vi "RemoteVI Translate Input.vi"(0 "kind":T2(ring), 1 "msg":u32, 2 "x":i32, 3 "y":i32, 4 "wParam":u64, 5 "lParam":i64, 6 "geo":T1, 7 "tracking in":bool, 8 "popup":bool) -> (20 "posts":cluster{"msg":u32, "wParam":u64, "lParam":i64}[](array[cluster]), 21 "tracking out":bool, 22 "cursor":cluster{"move?":bool, "x":i32, "y":i32})   [LabVIEW 2020, in "RemoteVI.lvlib"]
doc: "Turns one parsed client input message (the outputs of RemoteVI Parse Input.vi) into the Win32 messages the server posts to the panel window (docs/protocol.md section 4). Only the allowed messages of section 4.3 produce posts; anything else - ack, invalid, WM_CLOSE, WM_SYSKEYDOWN - gives an empty posts array and leaves tracking unchanged. WM_CHAR becomes three posts: WM_KEYDOWN(0xE8,1), WM_CHAR(wParam,1), WM_KEYUP(0xE8,0xC0000001). Other key messages pass through, except that a WM_KEYDOWN/WM_KEYUP whose lParam has no scan code (bits 16-23 zero - the browser client sends none) gets the key's set-1 scan code from the table below (LabVIEW lost the arrow key of a posted Shift + Right when both had scan code 0, measured). A double click (WM_xBUTTONDBLCLK) is posted as a second WM_xBUTTONDOWN: LabVIEW's panel window class has no CS_DBLCLKS, so Windows sends it two downs and LabVIEW ignores a posted DBLCLK (measured with a listbox Double Click event). Mouse lParam = ((y and 0xFFFF) shl 16) or (x and 0xFFFF) of CLIENT coordinates (screen point minus client origin) or of SCREEN coordinates (frame origin plus x/y - x and y are frame pixels, the frame being the window below its title bar): the wheel always uses screen; a button-down uses client and starts tracking; a button-up uses screen while tracking in is TRUE, else client, and ends tracking; a move uses screen while tracking in is TRUE, else client. The server passes as tracking in whether LabVIEW tracks the press right now - its UI thread holds the mouse capture (RemoteVI Mouse Captured.vi), read after LabVIEW handled the button-down. LabVIEW reads moves and the button-up as SCREEN coordinates only while it tracks (latched buttons, sliders, text selection, graph drags); a switch-when-pressed does not track and lost a screen-coordinate button-up (measured). While a LabVIEW popup is open (popup TRUE) only BUTTON messages are posted: with SCREEN coordinates, and cursor asks the caller to move the host cursor to that screen point just for the click (popup menus read the real cursor); tracking follows the same button rules. Moves and the wheel are DROPPED while a popup is open (no posts, tracking unchanged, no cursor), so the host cursor stays where the host user left it. Key messages are unaffected by popup. Pure function, cannot fail. Reference: translateInput() in tools\\lib\\input.mjs."
uses:
  RemoteVI.lvlib
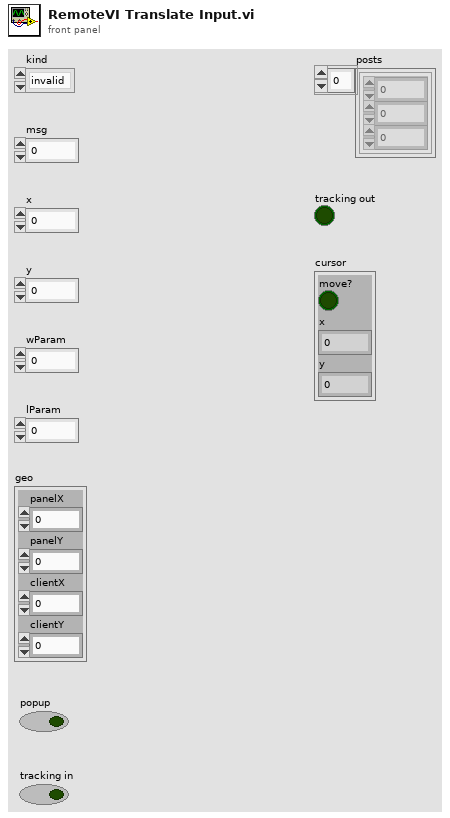
[diagram p1: front panel]
types:
  T1 = cluster{"panelX":i32, "panelY":i32, "clientX":i32, "clientY":i32}
  T2 = enum16{"invalid", "mouse", "key", "ack", "close", "splitter"}
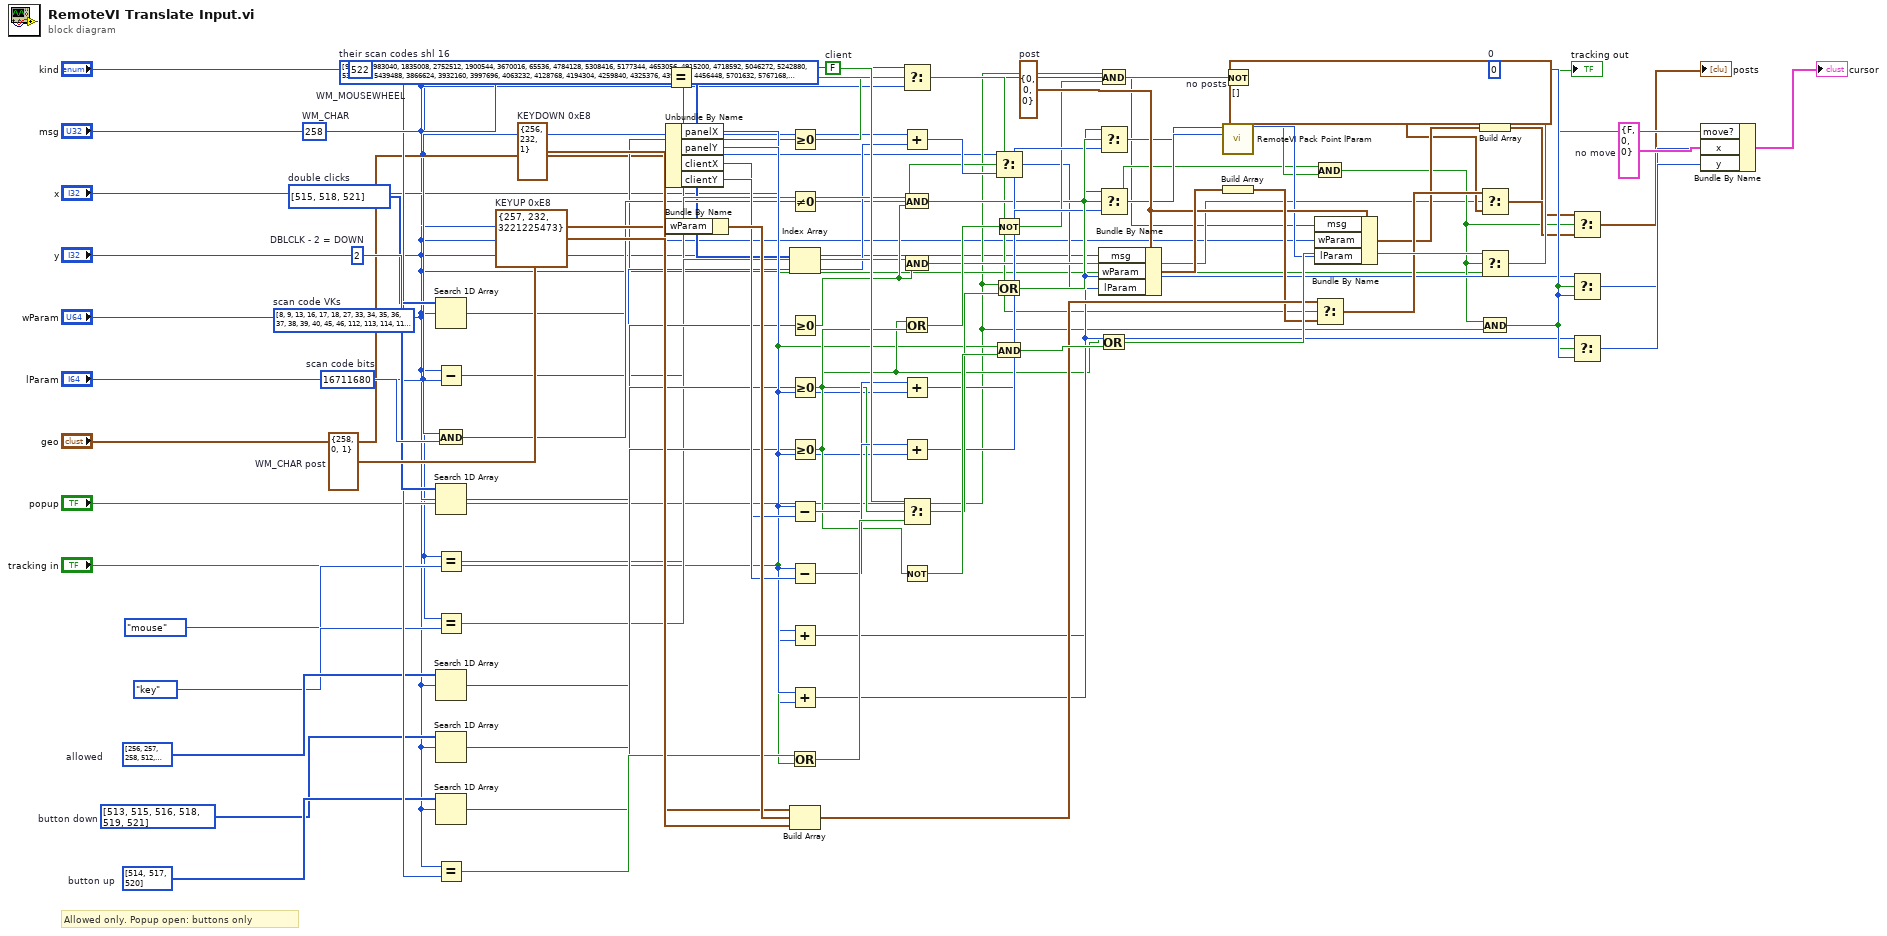
[diagram p0: block diagram]
diagram:
  w88 = cluster{"move?":bool, "x":i32, "y":i32} {"move?"=FALSE, "x"=0, "y"=0}  # no move
  w85 = 0  # 0
  w70 = cluster{"msg":u32, "wParam":u64, "lParam":i64}[] []  # no posts
  w69 = cluster{"msg":u32, "wParam":u64, "lParam":i64} {"msg"=257, "wParam"=232, "lParam"=3221225473}  # KEYUP 0xE8
  w68 = cluster{"msg":u32, "wParam":u64, "lParam":i64} {"msg"=256, "wParam"=232, "lParam"=1}  # KEYDOWN 0xE8
  w67 = cluster{"msg":u32, "wParam":u64, "lParam":i64} {"msg"=258, "wParam"=0, "lParam"=1}  # WM_CHAR post
  w66 = cluster{"msg":u32, "wParam":u64, "lParam":i64} {"msg"=0, "wParam"=0, "lParam"=0}  # post
  w59 = FALSE  # client
  w25 = i64 16711680  # scan code bits
  w24 = i64[] [917504, 983040, 1835008, 2752512, 1900544, 3670016, 65536, 4784128, 5308416, 5177344, 4653056, 4915200, 4718592, 5046272, 5242880, 5373952, 5439488, 3866624, 3932160, 3997696, 4063232, 4128768, 4194304, 4259840, 4325376, 4390912, 4456448, 5701632, 5767168, 2752512, 3538944, 1900544, 1900544, 3670016, 3670016]  # their scan codes shl 16
  w23 = u64[] [8, 9, 13, 16, 17, 18, 27, 33, 34, 35, 36, 37, 38, 39, 40, 45, 46, 112, 113, 114, 115, 116, 117, 118, 119, 120, 121, 122, 123, 160, 161, 162, 163, 164, 165]  # scan code VKs
  w18 = u32 2  # DBLCLK - 2 = DOWN
  w17 = u32[] [515, 518, 521]  # double clicks
  w16 = u32 258  # WM_CHAR
  w15 = u32 522  # WM_MOUSEWHEEL
  w14 = u32[] [514, 517, 520]  # button up
  w13 = u32[] [513, 515, 516, 518, 519, 521]  # button down
  w12 = u32[] [256, 257, 258, 512, 513, 514, 515, 516, 517, 518, 519, 520, 521, 522]  # allowed
  # "Allowed only. Popup open: buttons only"
  n1 = Search 1D Array(1D array=w17, element="msg") -> (index of element=w19:i32)  [unwired: 1 in]
  n2 = Subtract(x="msg", y=w18) -> (x-y=w21:u32)
  n3 = And(x="lParam", y=w25) -> (x .and. y?=w26:i64)
  n4 = Search 1D Array(1D array=w23, element="wParam") -> (index of element=w28:i32)  [unwired: 1 in]
  n5 = Equal?(x="kind", y=T2."mouse") -> (x = y?=w32:bool)
  n6 = Equal?(x="kind", y=T2."key") -> (x = y?=w33:bool)
  n7 = Search 1D Array(1D array=w12, element="msg") -> (index of element=w34:i32)  [unwired: 1 in]
  n8 = Search 1D Array(1D array=w13, element="msg") -> (index of element=w35:i32)  [unwired: 1 in]
  n9 = Search 1D Array(1D array=w14, element="msg") -> (index of element=w36:i32)  [unwired: 1 in]
  n10 = Equal?(x="msg", y=w15) -> (x = y?=w40:bool)
  n11 = Equal?(x="msg", y=w16) -> (x = y?=w41:bool)
  n12 = Unbundle By Name("geo") -> ("panelX"=w49:i32, "panelY"=w50:i32, "clientX"=w51:i32, "clientY"=w52:i32)
  n13 = Bundle By Name(cluster=w67, "wParam"="wParam") -> (w75:cluster{"msg":u32, "wParam":u64, "lParam":i64})
  n14 = Greater Or Equal To 0?(x=w19) -> (x >= 0?=w20:bool)
  n15 = Not Equal To 0?(x=w26) -> (x != 0?=w27:bool)
  n16 = Index Array(array=w24, index=w28) -> (element=w29:i64)
  n17 = Greater Or Equal To 0?(x=w34) -> (x >= 0?=w37:bool)
  n18 = Greater Or Equal To 0?(x=w35) -> (x >= 0?=w38:bool)
  n19 = Greater Or Equal To 0?(x=w36) -> (x >= 0?=w39:bool)
  n20 = Subtract(x=w49, y=w51) -> (x-y=w53:i32)
  n21 = Subtract(x=w50, y=w52) -> (x-y=w54:i32)
  n22 = Add(x=w49, y="x") -> (x+y=w55:i32)
  n23 = Add(x=w50, y="y") -> (x+y=w56:i32)
  n24 = Or(x=w40, y="tracking in") -> (x .or. y?=w60:bool)
  n25 = Build Array(w68, w75, w69) -> (w76:cluster{"msg":u32, "wParam":u64, "lParam":i64}[])
  n26 = Select(t=w21, s=w20, f="msg") -> (s? t:f=w22:u32)
  n27 = Add(x="lParam", y=w29) -> (x+y=w30:i64)
  n28 = And(x=w32, y=w37) -> (x .and. y?=w42:bool)
  n29 = And(x=w33, y=w37) -> (x .and. y?=w43:bool)
  n30 = Or(x=w38, y=w39) -> (x .or. y?=w44:bool)
  n31 = Add(x=w53, y="x") -> (x+y=w57:i32)
  n32 = Add(x=w54, y="y") -> (x+y=w58:i32)
  n33 = Select(t=w59, s=w38, f=w60) -> (s? t:f=w61:bool)
  n34 = Not(x=w39) -> (.not. x?=w80:bool)
  n35 = Select(t="lParam", s=w27, f=w30) -> (s? t:f=w31:i64)
  n36 = Not(x=w44) -> (.not. x?=w45:bool)
  n37 = Or(x="popup", y=w61) -> (x .or. y?=w62:bool)
  n38 = And(x="tracking in", y=w80) -> (x .and. y?=w81:bool)
  n39 = And(x="popup", y=w45) -> (x .and. y?=w46:bool)
  n40 = Select(t=w55, s=w62, f=w57) -> (s? t:f=w63:i32)
  n41 = Select(t=w56, s=w62, f=w58) -> (s? t:f=w64:i32)
  n42 = Bundle By Name(cluster=w66, "msg"="msg", "wParam"="wParam", "lParam"=w31) -> (w73:cluster{"msg":u32, "wParam":u64, "lParam":i64})
  n43 = Or(x=w38, y=w81) -> (x .or. y?=w82:bool)
  n44 = Not(x=w46) -> (.not. x?=w47:bool)
  n45 = call "RemoteVI Pack Point lParam.vi"("x"=w63, "y"=w64) -> ("lParam"=w65:i64)  [unwired: 13 in]
  n46 = Build Array(w73) -> (w74:cluster{"msg":u32, "wParam":u64, "lParam":i64}[])
  n47 = And(x=w42, y=w47) -> (x .and. y?=w48:bool)
  n48 = Bundle By Name(cluster=w66, "msg"=w22, "wParam"="wParam", "lParam"=w65) -> (w71:cluster{"msg":u32, "wParam":u64, "lParam":i64})
  n49 = Select(t=w76, s=w41, f=w74) -> (s? t:f=w77:cluster{"msg":u32, "wParam":u64, "lParam":i64}[])
  n50 = Build Array(w71) -> (w72:cluster{"msg":u32, "wParam":u64, "lParam":i64}[])
  n51 = Select(t=w77, s=w43, f=w70) -> (s? t:f=w78:cluster{"msg":u32, "wParam":u64, "lParam":i64}[])
  n52 = Select(t=w82, s=w48, f="tracking in") -> (s? t:f=→"tracking out":bool)
  n53 = And(x=w48, y="popup") -> (x .and. y?=w84:bool)
  n54 = Select(t=w72, s=w48, f=w78) -> (s? t:f=→"posts":cluster{"msg":u32, "wParam":u64, "lParam":i64}[])
  n55 = Select(t=w55, s=w84, f=w85) -> (s? t:f=w86:i32)
  n56 = Select(t=w56, s=w84, f=w85) -> (s? t:f=w87:i32)
  n57 = Bundle By Name(cluster=w88, "move?"=w84, "x"=w86, "y"=w87) -> (→"cursor":cluster{"move?":bool, "x":i32, "y":i32})
